vi "boolean.vi"(11 "input":bool) -> (3 "output":bool=TRUE)   [LabVIEW 2021]
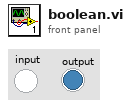
[diagram p1: front panel]
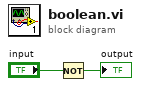
[diagram p0: block diagram]
diagram:
  n1 = Not(x="input") -> (.not. x?=→"output":bool)
